vi "Pre Launch Init.vi"(11 "ImageHandler:Varex-ImageHandler in":refnum<class "Varex-ImageHandler.lvclass">) -> (0 "error out":errorcluster, 3 "ImageHandler:Varex-ImageHandler out":refnum<class "Varex-ImageHandler.lvclass">)   [LabVIEW 2022 SP3, in "ImageHandler.lvlib" / "Varex-ImageHandler.lvclass"]
doc: "(<B>Filename</B>: Actor Framework.lvlib:Actor.lvclass:Pre Launch Init.vi)\n\nDefines behavior that occurs after the Launch Actor method is invoked but before the actor's Actor Core method begins running.\n\nThe Pre Launch Init method is guaranteed to finish before the Launch Actor method returns to its caller and before the actor itself receives any messages. Any references that the Pre Launch Init method obtains are guaranteed to have the same lifetime as the actor itself. Any errors that the Pre Launch Init method returns will abort the launch.\n\nBy default, this method does nothing. A descendant class may override it to define behavior."
uses:
  Varex-ImageHandler.lvclass
  Varex-ImageHandler.lvclass/Varex-ImageHandler.ctl
  ImageHandler/ImageHandler.lvclass
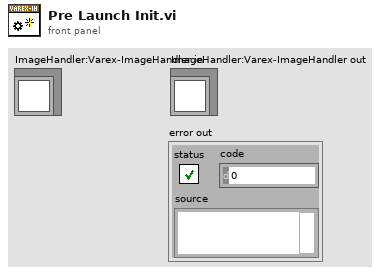
[diagram p1: front panel]
types:
  T1 = typedef "Image Type" = u32
  T2 = typedef "IMAQ Image.ctl" = refnum<image>
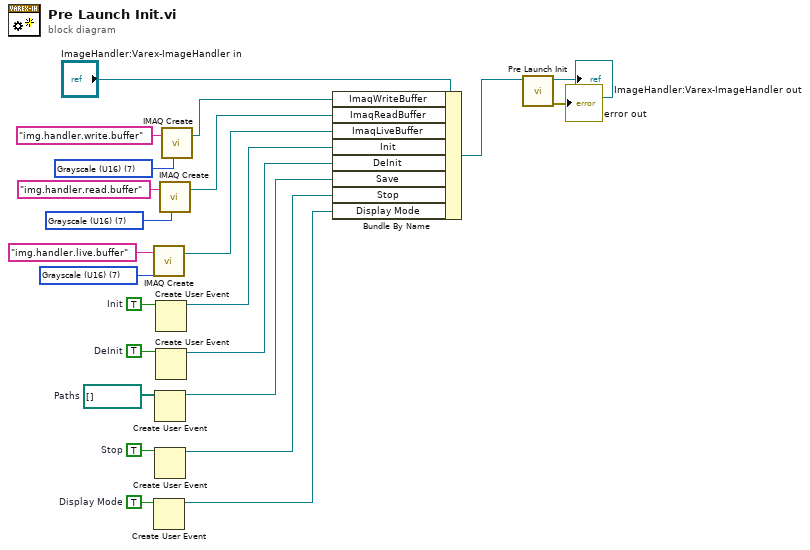
[diagram p0: block diagram]
diagram:
  w2 = TRUE  # Display Mode
  w4 = T1 7 items=["Grayscale (U8)", "Grayscale (I16)", "Grayscale (SGL)", "Complex (CSG)", "RGB (U32)", "HSL (U32)", "RGB (U64)", "Grayscale (U16)"] ("Image Type")
  w10 = TRUE  # Stop
  w11 = path[] []  # Paths
  w12 = TRUE  # DeInit
  w13 = TRUE  # Init
  w16 = T1 7 items=["Grayscale (U8)", "Grayscale (I16)", "Grayscale (SGL)", "Complex (CSG)", "RGB (U32)", "HSL (U32)", "RGB (U64)", "Grayscale (U16)"] ("Image Type")
  w17 = T1 7 items=["Grayscale (U8)", "Grayscale (I16)", "Grayscale (SGL)", "Complex (CSG)", "RGB (U32)", "HSL (U32)", "RGB (U64)", "Grayscale (U16)"] ("Image Type")
  n1 = call "IMAQ Create"("Image Name"="img.handler.live.buffer", "Image Type"=w4) -> ("New Image"=w3:T2)  [unwired: 3 in, 1 out]
  n2 = Create User Event(user event datatype=w2) -> (user event=w1:refnum<user-event>)  [unwired: 1 in, 1 out]
  n3 = Create User Event(user event datatype=w11) -> (user event=w7:refnum<user-event>)  [unwired: 1 in, 1 out]
  n4 = Create User Event(user event datatype=w10) -> (user event=w6:refnum<user-event>)  [unwired: 1 in, 1 out]
  n5 = Create User Event(user event datatype=w13) -> (user event=w9:refnum<user-event>)  [unwired: 1 in, 1 out]
  n6 = Create User Event(user event datatype=w12) -> (user event=w8:refnum<user-event>)  [unwired: 1 in, 1 out]
  n7 = call "IMAQ Create"("Image Name"="img.handler.read.buffer", "Image Type"=w16) -> ("New Image"=w15:T2)  [unwired: 3 in, 1 out]
  n8 = call "IMAQ Create"("Image Name"="img.handler.write.buffer", "Image Type"=w17) -> ("New Image"=w14:T2)  [unwired: 3 in, 1 out]
  n9 = Bundle By Name(cluster="ImageHandler:Varex-ImageHandler in", "ImaqWriteBuffer"=w14, "ImaqReadBuffer"=w15, "ImaqLiveBuffer"=w3, "Init"=w9, "DeInit"=w8, "Save"=w7, "Stop"=w6, "Display Mode"=w1) -> (w20:refnum<class "Varex-ImageHandler.lvclass">)
  n10 = call-parent "Pre Launch Init.vi"("ImageHandler in"=w20) -> ("error out"=→"error out":errorcluster, "ImageHandler out"=→"ImageHandler:Varex-ImageHandler out":refnum<class "Varex-ImageHandler.lvclass">)  [unwired: 9 in]
